vi "Build CE Deploy - List Files.vi"(6 "Exclude file names":string, 8 "error in":errorcluster, 9 "Exclude undesired paths (F)":bool, 10 "Folders":string, 11 "Source Dir":path) -> (0 "error out":errorcluster, 1 "Files to Copy":path[](array[path]), 2 "Project Files":path[](array[path]), 3 "dup Source Dir":path, 5 "Excluded Paths":path[](array[path]))   [LabVIEW 2021]
doc: "::: CalcExpress Toolkit :::\nCopyright (c) 2000-2026 Konstantin Shifershteyn. All rights reserved."
uses:
  <vilib>/Utility/lvfile.llb/NI_FileType.lvlib
panel:
  # "CalcExpress Toolkit\nCopyright (c) 2000-2026 Konstantin Shifershteyn"
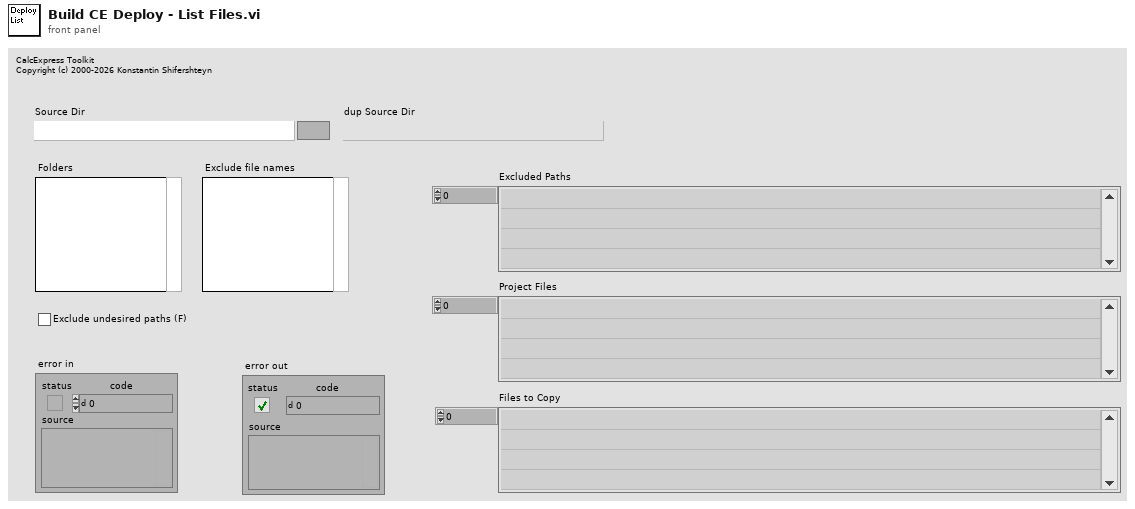
[diagram p1: front panel]
types:
  T1 = typedef "NI_FileType.lvlib/FT_FileTypes.ctl" = enum32{"Invalid file/path", "Unknown type", "Instrument", "Control", "Polymorphic VI", "Project", "Library", "LVClass", "XControl", "XNode", "CIN", "Run-time menu", "Palette menu", "LLB", "Shortcut", "Directory", "Class Private Data Control", "Statechart", "MathScript .m file", "Ladder Diagram", "LVLibp"}
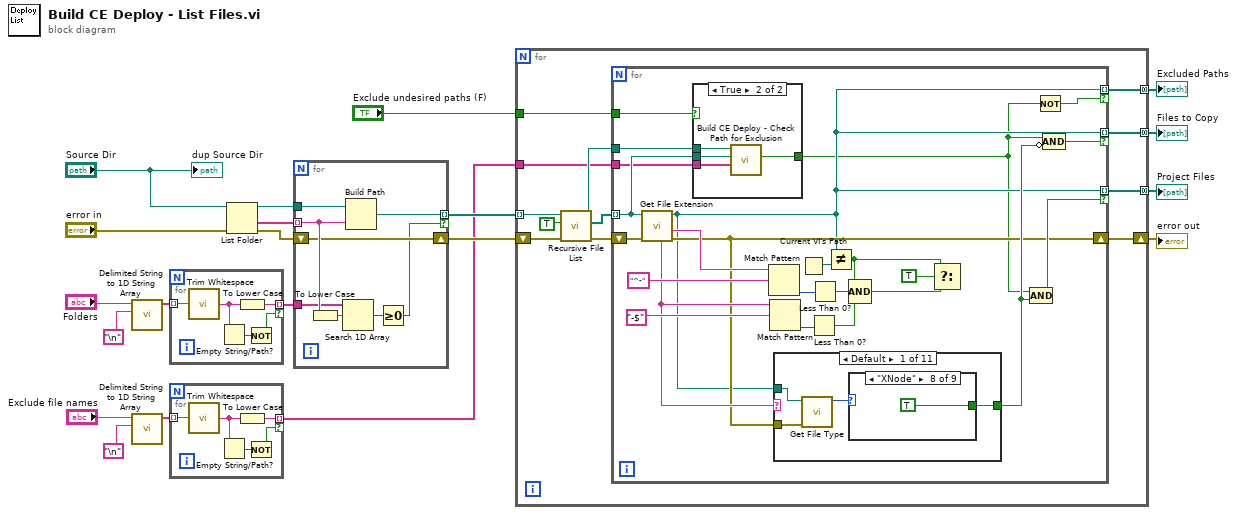
[diagram p0: block diagram]
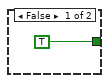
[diagram p2: hidden frame]
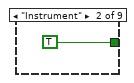
[diagram p4: hidden frame]
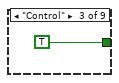
[diagram p5: hidden frame]
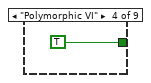
[diagram p6: hidden frame]
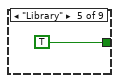
[diagram p7: hidden frame]
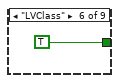
[diagram p8: hidden frame]
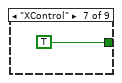
[diagram p9: hidden frame]
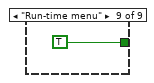
[diagram p10: hidden frame]
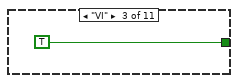
[diagram p12: hidden frame]
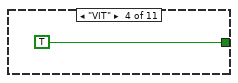
[diagram p13: hidden frame]
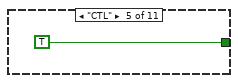
[diagram p14: hidden frame]
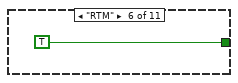
[diagram p15: hidden frame]
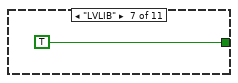
[diagram p16: hidden frame]
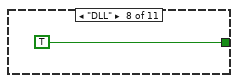
[diagram p17: hidden frame]
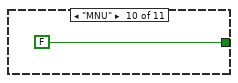
[diagram p19: hidden frame]
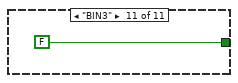
[diagram p20: hidden frame]
diagram:
  n1 = call <vilib>:"Delimited String to 1D String Array.vi"("delimiter"="\n", "delimited string"="Folders") -> ("string array"=w18:string[])  [unwired: 9 in]
  n2 = call <vilib>:"Delimited String to 1D String Array.vi"("delimiter"="\n", "delimited string"="Exclude file names") -> ("string array"=w4:string[])  [unwired: 9 in]
  n3 = for {
    tunnel: w18 -> [w25] mode=indexing
    tunnel: [w21] -> w15 mode=indexing if=w22
    n4 = call <vilib>:"Trim Whitespace.vi"("string"=w25) -> ("trimmed string"=w24:string)  [unwired: 1 in]
    n5 = Empty String/Path?(string/path=w24) -> (empty?=w23:bool)
    n6 = To Lower Case(string=w24) -> (all lower case string=w21:string)
    n7 = Not(x=w23) -> (.not. x?=w22:bool)
  }
  n8 = for {
    tunnel: w4 -> [w30] mode=indexing
    tunnel: [w26] -> w1 mode=indexing if=w27
    n9 = call <vilib>:"Trim Whitespace.vi"("string"=w30) -> ("trimmed string"=w29:string)  [unwired: 1 in]
    n10 = Empty String/Path?(string/path=w29) -> (empty?=w28:bool)
    n11 = To Lower Case(string=w29) -> (all lower case string=w26:string)
    n12 = Not(x=w28) -> (.not. x?=w27:bool)
  }
  n13 = List Folder(path="Source Dir", error in="error in") -> (path out=w14:path, folder names=w16:string[], error out=w12:errorcluster)  [unwired: 2 in, 1 out]
  n14 = for {
    tunnel: w16 -> [w37] mode=indexing
    tunnel: w15 -> [w31]
    tunnel: w14 -> [w38]
    tunnel: [w36] -> w13 mode=indexing if=w32
    shift-right: [w35] -> w11
    shift-left: w12 -> [w35]
    n15 = To Lower Case(string=w37) -> (all lower case string=w34:string)
    n16 = Search 1D Array(1D array=w31, element=w34) -> (index of element=w33:i32)  [unwired: 1 in]
    n17 = Build Path(base path=w38, name or relative path=w37) -> (appended path=w36:path)
    n18 = Greater Or Equal To 0?(x=w33) -> (x >= 0?=w32:bool)
  }
  n19 = for {
    tunnel: w13 -> [w47] mode=indexing
    shift-right: [w45] -> w8
    shift-left: w11 -> [w46]
    tunnel: [w44] -> w9 mode=concatenating
    tunnel: [w43] -> w10 mode=concatenating
    tunnel: "Exclude undesired paths (F)" -> [w41]
    tunnel: [w40] -> w5 mode=concatenating
    tunnel: w1 -> [w39]
    n20 = call <vilib>:"Recursive File List.vi"("error in (no error)"=w46, "Treat LLBs as Folders?"=TRUE, "Folder Path"=w47) -> ("error out"=w50:errorcluster, "All Files in Dir"=w48:path[], "dup Folder Path"=w42:path)  [unwired: 4 in, 2 out]
    n21 = for {
      tunnel: w48 -> [w57] mode=indexing
      tunnel: [w54] -> w44 mode=indexing if=w66
      shift-right: [w61] -> w45
      shift-left: w50 -> [w65]
      tunnel: [w54] -> w43 mode=indexing if=w62
      tunnel: w42 -> [w56]
      tunnel: w41 -> [w55]
      tunnel: [w54] -> w40 mode=indexing if=w52
      tunnel: w39 -> [w51]
      n22 = call <vilib>:"Get File Extension.vi"("error in (no error)"=w65, "file"=w57) -> ("error out"=w61:errorcluster, "filename without extension"=w74:string, "dup file"=w54:path, "unmodified file extension"=w69:string)  [unwired: 5 in, 1 out]
      n23 = case shown="True" w55 {
        tunnel: w57 -> [_ w79]
        tunnel: w56 -> [_ w78]
        tunnel: [TRUE w77] -> w53
        tunnel: w51 -> [_ w76]
        frame False {
        }
        frame True {
          n24 = call "Build CE Deploy - Check Path for Exclusion.vi"("Exclude file name patterns"=w76, "Path"=w79, "Base dir"=w78) -> ("pass"=w77:bool)  [unwired: 8 in]
        }
      }
      n25 = Match Pattern(string=w74, regular expression="^-") -> (offset past match=w71:i32)  [unwired: 1 in, 3 out]
      n26 = Match Pattern(string=w69, regular expression="-$") -> (offset past match=w72:i32)  [unwired: 1 in, 3 out]
      n27 = case shown="Default" w69 {
        tunnel: [w81 _ TRUE TRUE TRUE TRUE TRUE TRUE _ FALSE FALSE] -> w63
        tunnel: w54 -> [w83 _ _ _ _ _ _ _ _ _ _]
        tunnel: w61 -> [w80 _ _ _ _ _ _ _ _ _ _]
        frame Default {
          n28 = call <vilib>:"Get File Type.vi"("error in (no error)"=w80, "path"=w83) -> ("file type"=w82:T1)  [unwired: 7 in, 2 out]
          n29 = case shown="\"XNode\"" w82 {
            tunnel: [_ TRUE TRUE TRUE TRUE TRUE TRUE TRUE TRUE] -> w81
            frame Default {
            }
            frame "Instrument" {
            }
            frame "Control" {
            }
            frame "Polymorphic VI" {
            }
            frame "Library" {
            }
            frame "LVClass" {
            }
            frame "XControl" {
            }
            frame "XNode" {
            }
            frame "Run-time menu" {
            }
          }
        }
        frame "----- 1" {
        }
        frame "VI" {
        }
        frame "VIT" {
        }
        frame "CTL" {
        }
        frame "RTM" {
        }
        frame "LVLIB" {
        }
        frame "DLL" {
        }
        frame "----- 2" {
        }
        frame "MNU" {
        }
        frame "BIN3" {
        }
      }
      n30 = Current VI's Path() -> (path=w64:path)
      n31 = Less Than 0?(x=w72) -> (x < 0?=w67:bool)
      n32 = Less Than 0?(x=w71) -> (x < 0?=w68:bool)
      n33 = Not Equal?(x=w54, y=w64) -> (x != y?=w60:bool)
      n34 = Compound Arithmetic op=AND(w60, w68, w67) -> (w59:bool)
      n35 = Select(t=w60, s=TRUE, f=w59) -> ()  [unwired: 1 out]
      n36 = Compound Arithmetic op=AND(w53, w63) -> (w66:bool)
      n37 = Not(x=w53) -> (.not. x?=w52:bool)
      n38 = Compound Arithmetic op=AND(w53, invert w63) -> (w62:bool)
    }
  }
  "error out" <- w8
  "Project Files" <- w9
  "Files to Copy" <- w10
  "Excluded Paths" <- w5
  "dup Source Dir" <- "Source Dir"
